vi "Read Input and Output Config File.vi"(8 "error in (no error)":errorcluster) -> (0 "error out":errorcluster, 3 "Input and Output Settings":T1[](array[typedef]))   [LabVIEW 2021]
uses:
  TypeDefs/Device Settings.ctl
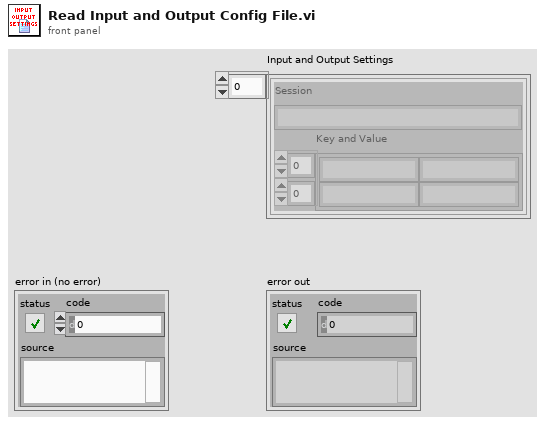
[diagram p1: front panel]
types:
  T1 = typedef "Device Settings.ctl" = cluster{"Session":string, "Key and Value":string[][]}
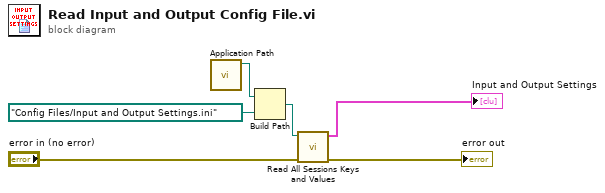
[diagram p0: block diagram]
diagram:
  n1 = call "Application Path.vi"() -> ("appended path"=w6:path)  [unwired: 11 in]
  n2 = Build Path(base path=w6, name or relative path=path "Config Files/Input and Output Settings.ini" ("configuration file path")) -> (appended path=w4:path)
  n3 = call "Read All Sessions Keys and Values.vi"("error in (no error)"="error in (no error)", "appended path"=w4) -> ("error out"=→"error out":errorcluster, "Device Settings"=→"Input and Output Settings":T1[])  [unwired: 8 in]
